vi "Diagnostics Message Loop.vi"(8 "error in (no error)":errorcluster, 11 "Message Queues":T1) -> (0 "error out":errorcluster)   [LabVIEW 2021, in "Diagnostics.lvlib"]
doc: "Message loop for handling messages pertaining to logging information to a debug log file."
uses:
  Diagnostics.lvlib
  support/Message Queue/All Message Queues.ctl
  support/Message Queue/Message Cluster.ctl
  Diagnostics State.ctl
  <vilib>/Utility/error.llb/Error Cluster From Error Code.vi
  <vilib>/ErrorRing/Error Ring.xnode
  support/Message Queue/Message Queue.lvlib
  Settings/Settings.lvlib
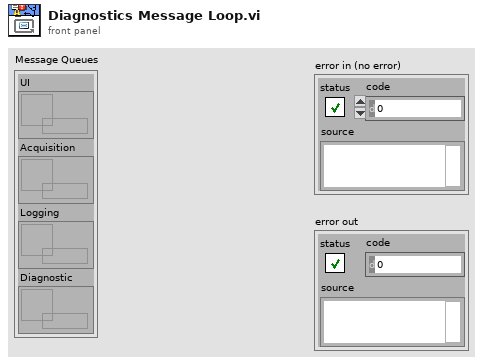
[diagram p1: front panel]
types:
  T1 = typedef "Message Queue.lvlib/All Message Queues.ctl" = cluster{"UI":refnum<queue>, "Acquisition":refnum<queue>, "Logging":refnum<queue>, "Diagnostic":refnum<queue>}
  T2 = typedef "Diagnostics.lvlib/Diagnostics State.ctl" = enum16{"Idle", "Active"}
  T3 = typedef "Settings.lvlib/Settings.ctl" = cluster{"IO":T4, "Log":T10, "Debug":T11}
  T4 = typedef "Acquisition.lvlib/Hardware Configuration.ctl" = cluster{"Channel Settings":T5[], "Sensor Intervals":T7[], "Sensor Token":T9}
  T5 = typedef "Acquisition.lvlib/Channel Settings.ctl" = cluster{"Name":string, "Terminal Information":cluster{"IO Device":T6, "Channel Number":i32}, "Calibration Information":cluster{"Excitation Voltage":dbl, "Calibration Factor":dbl, "Zero Value":dbl, "Calibration Formula":string}}
  T6 = typedef "Acquisition.lvlib/IO Device.ctl" = enum16{"none", "9219", "9401"}
  T7 = typedef "Interval Timer.lvlib/Repeat Interval.ctl" = cluster{"Interval":T8, "Count":i32}
  T8 = typedef "Interval Timer.lvlib/Interval Length.ctl" = enum16{"Manual control", "1 second", "10 seconds", "30 seconds", "60 seconds", "600 seconds", "1200 seconds", "3600 seconds"}
  T9 = typedef "Interval Timer.lvlib/Interval Token.ctl" = cluster{"Next reading in ms":u32, "Interval Index":i32, "Interval Occurrence":i32}
  T10 = typedef "Logging.lvlib/Logging Configuration.ctl" = cluster{"Path":path, "Spreadsheet":refnum<file>, "Append":bool}
  T11 = typedef "Diagnostics.lvlib/Diagnostics Configuration.ctl" = cluster{"Messages":refnum<file>}
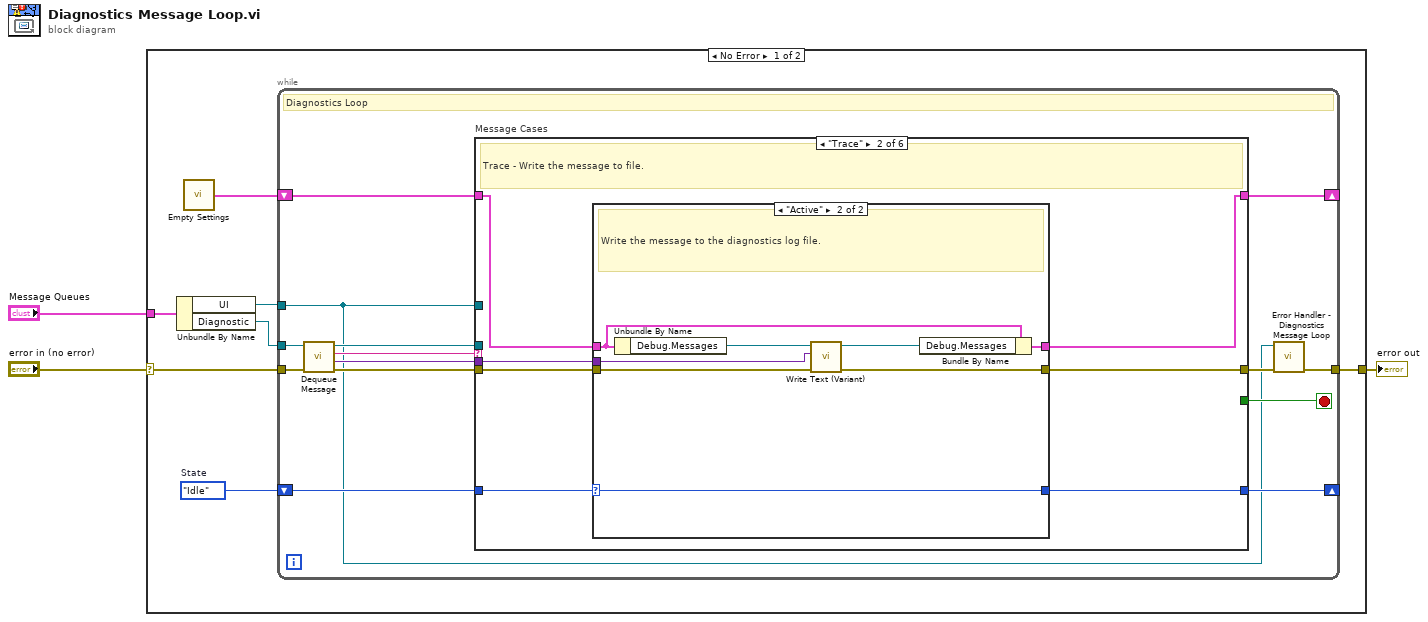
[diagram p0: block diagram]
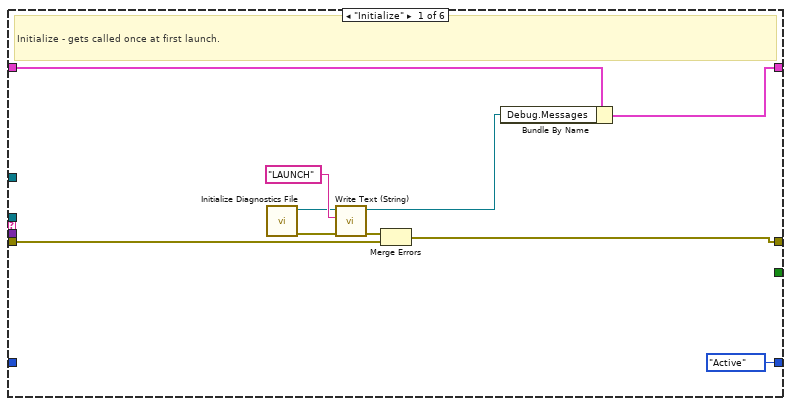
[diagram p2: hidden frame]
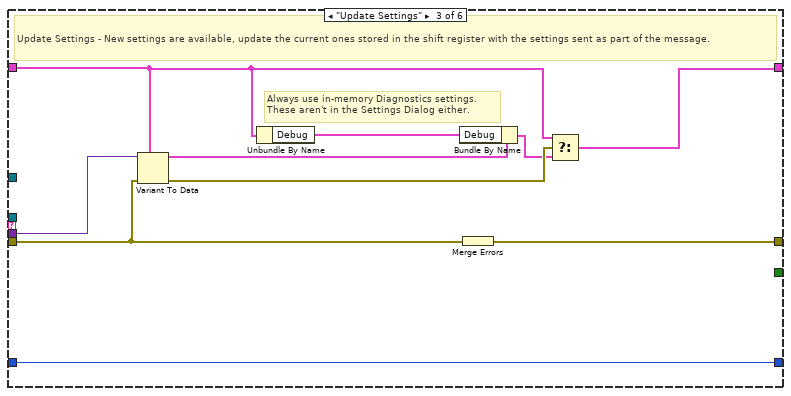
[diagram p4: hidden frame]
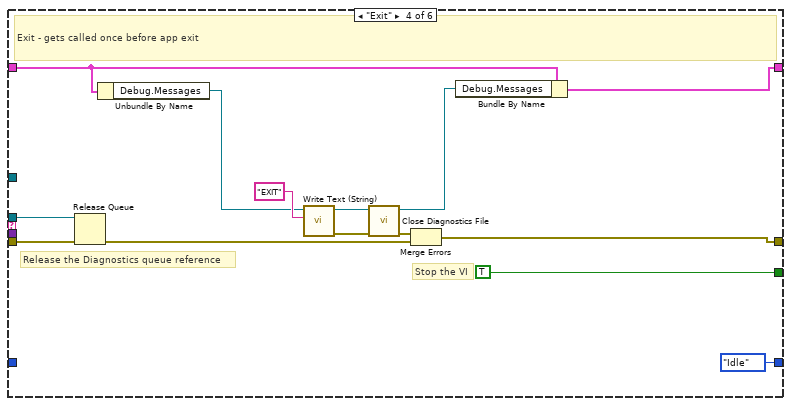
[diagram p5: hidden frame]
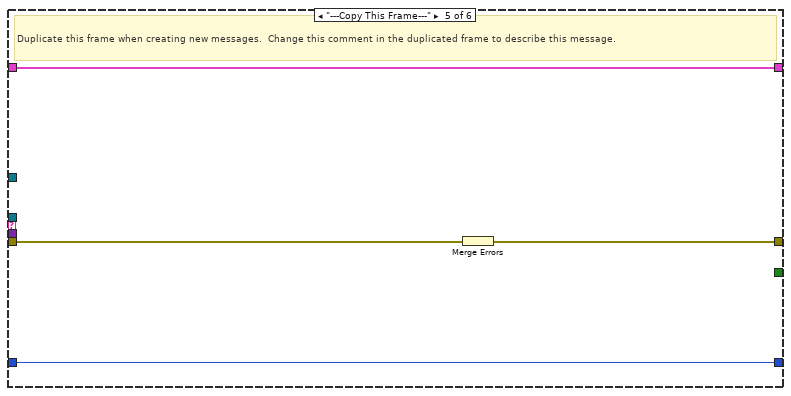
[diagram p6: hidden frame]
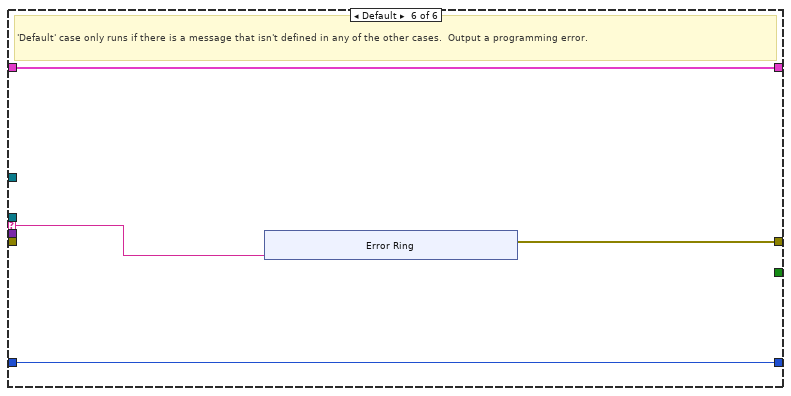
[diagram p7: hidden frame]
diagram:
  n1 = case shown="No Error" "error in (no error)" {
    selector: "error in (no error)" -> [w7 w92]
    tunnel: "Message Queues" -> [w10 _]
    tunnel: [w8 w92] -> w2
    frame No Error {
      w5 = Diagnostics_State."Idle"  # State
      n2 = Unbundle By Name(w10) -> ("UI"=w6:refnum<queue>, "Diagnostic"=w9:refnum<queue>)
      n3 = call "Empty Settings.vi"() -> ("Settings"=w4:T3)
      n4 = while {
        tunnel: w9 -> [w16]
        shift-right: [w23] -> _
        shift-left: w4 -> [w24]
        tunnel: w6 -> [w11]
        shift-right: [w14] -> _
        shift-left: w5 -> [w15]
        tunnel: w7 -> [w21]
        tunnel: [w13] -> w8
        stop <- w22 stop-if-true
        # "Diagnostics Loop"
        n5 = call "Dequeue Message.vi"("error in (no error)"=w21, "Message Queue"=w16) -> ("error out"=w20:errorcluster, "Message Data"=w18:variant, "Message"=w19:string, "dup Message Queue"=w17:refnum<queue>)  [unwired: 6 in]
        n6 = case "Message Cases" shown="\"Trace\"" w19 {
          selector: w19 -> [_ _ _ _ _ w81]
          tunnel: w17 -> [_ _ _ w73 _ _]
          tunnel: w20 -> [w33 w40 w58 w74 w80 _]
          tunnel: [w32 w41 w62 w75 w78 w82] -> w12
          tunnel: w24 -> [w34 w36 w56 w71 w79 w84]
          tunnel: [w31 w35 w59 w70 w79 w84] -> w23
          tunnel: [_ _ _ TRUE _ _] -> w22
          tunnel: w18 -> [_ w37 w61 _ _ _]
          tunnel: w11 -> [_ _ _ _ _ _]
          tunnel: w15 -> [_ w39 w57 _ w77 w83]
          tunnel: [Diagnostics_State."Active" ("State") w38 w57 Diagnostics_State."Idle" ("State") w77 w83] -> w14
          frame "Initialize" {
            # "Initialize - gets called once at first launch."
            n7 = call "Initialize Diagnostics File.vi"() -> ("error out"=w30:errorcluster, "diagnostics file"=w27:refnum<file>)  [unwired: 10 in]
            n8 = call "Write Text (String).vi"("error in"=w30, "String"="LAUNCH" ("message"), "file in"=w27) -> ("error out"=w29:errorcluster, "file out"=w26:refnum<file>)  [unwired: 7 in]
            n9 = Merge Errors(w29, w33) -> (w32:errorcluster)
            n10 = Bundle By Name(cluster=w34, "Debug.Messages"=w26) -> (w31:T3)
          }
          frame "Trace" {
            # "Trace - Write the message to file."
            n11 = case shown="\"Active\"" w39 {
              selector: w39 -> [w44 w52]
              tunnel: [w43 w50] -> w41
              tunnel: w40 -> [w43 w51]
              tunnel: [w44 w52] -> w38
              tunnel: w37 -> [_ w49]
              tunnel: w36 -> [w42 w47]
              tunnel: [w42 w45] -> w35
              frame "Idle" {
                # "Ignore \"Trace\" messages when idle."
              }
              frame "Active" {
                # "Write the message to the diagnostics log file."
                n12 = Unbundle By Name(w47) -> ("Debug.Messages"=w48:refnum<file>)
                n13 = call "Write Text (Variant).vi"("error in"=w51, "Anything"=w49, "file in"=w48) -> ("error out"=w50:errorcluster, "file out"=w46:refnum<file>)  [unwired: 7 in]
                n14 = Bundle By Name(cluster=w47, "Debug.Messages"=w46) -> (w45:T3)
              }
            }
          }
          frame "Update Settings" {
            # "Always use in-memory Diagnostics settings.\nThese aren't in the Settings Dialog either."
            # "Update Settings - New settings are available, update the current ones stored in the shift register with the settings sent as part of the message."
            n15 = Variant To Data(error in=w58, type=w56, Variant=w61) -> (data=w54:T3, error out=w60:errorcluster)
            n16 = Unbundle By Name(w56) -> ("Debug"=w55:T11)
            n17 = Bundle By Name(cluster=w54, "Debug"=w55) -> (w53:T3)
            n18 = Merge Errors(w58) -> (w62:errorcluster)
            n19 = Select(t=w56, s=w60, f=w53) -> (s? t:f=w59:T3)
          }
          frame "Exit" {
            # "Release the Diagnostics queue reference"
            # "Stop the VI"
            # "Exit - gets called once before app exit"
            n20 = Release Queue(queue=w73, error in (no error)=w74) -> (error out=w68:errorcluster)  [unwired: 1 in, 2 out]
            n21 = Unbundle By Name(w71) -> ("Debug.Messages"=w65:refnum<file>)
            n22 = call "Write Text (String).vi"("String"="EXIT" ("message"), "file in"=w65) -> ("error out"=w67:errorcluster, "file out"=w64:refnum<file>)  [unwired: 8 in]
            n23 = call "Close Diagnostics File.vi"("error in"=w67, "diagnostics file"=w64) -> ("error out"=w69:errorcluster, "not a file refnum"=w72:refnum<file>)  [unwired: 8 in]
            n24 = Merge Errors(w69, w68) -> (w75:errorcluster)
            n25 = Bundle By Name(cluster=w71, "Debug.Messages"=w72) -> (w70:T3)
          }
          frame "---Copy This Frame---" {
            # "Duplicate this frame when creating new messages.  Change this comment in the duplicated frame to describe this message."
            n26 = Merge Errors(w80) -> (w78:errorcluster)
          }
          frame Default {
            # "'Default' case only runs if there is a message that isn't defined in any of the other cases.  Output a programming error."
            n27 = xnode "Error Ring"("parameter 0"=w81) -> ("error out"=w82:errorcluster)
          }
        }
        n28 = call "Error Handler - Diagnostics Message Loop.vi"("error in (no error)"=w12, "Message Queue"=w11) -> ("dup error in"=w13:errorcluster)  [unwired: 8 in, 1 out]
      }
    }
    frame Error {
    }
  }
  "error out" <- w2
